vi "Shorten Path for Display.vi"(10 "Keep":i32=3, 11 "Path":path) -> (3 "Shortened Path":path)   [LabVIEW 2026]
doc: "This VI shortens the provided path to ... followed by the number of levels specified by <i>keep</i>."
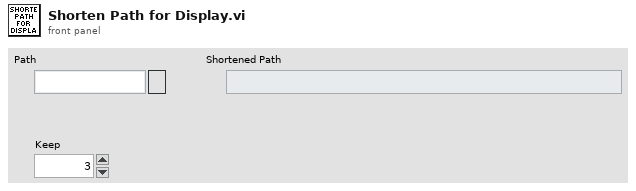
[diagram p1: front panel]
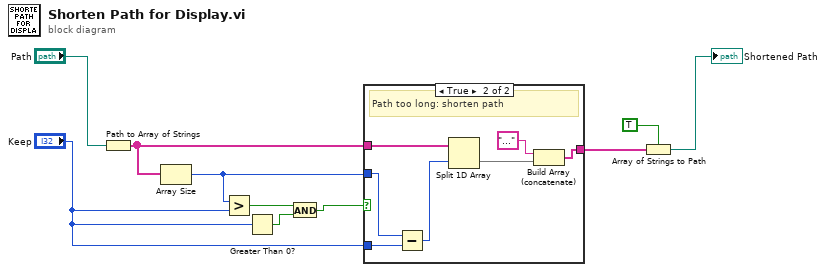
[diagram p0: block diagram]
diagram:
  n1 = Path to Array of Strings(0:"Path") -> (2:w8:string[])  [unwired: 1 out]
  n2 = Array Size(array=w8) -> (size(s)=w7:i32)
  n3 = Greater?(x=w7, y="Keep") -> (0:w9:bool)
  n4 = Greater Than 0?(x="Keep") -> (x > 0?=w2:bool)
  n5 = And(x=w9, y=w2) -> (x .and. y?=w3:bool)
  n6 = case shown="True" w3 {
    tunnel: w8 -> [w11 w18]
    tunnel: w7 -> [_ w17]
    tunnel: "Keep" -> [_ w16]
    tunnel: [w11 w12] -> w6
    frame False {
      # "Path short enough"
    }
    frame True {
      # "Path too long: shorten path"
      n7 = Subtract(x=w17, y=w16) -> (x-y=w15:i32)
      n8 = Split 1D Array(array=w18, index=w15) -> (second subarray=w14:string[])  [unwired: 1 out]
      n9 = Build Array (concatenate)("...", w14) -> (w12:string[])
    }
  }
  n10 = Array of Strings to Path(0:w6, 1:TRUE ("relative")) -> (2:→"Shortened Path":path)
